vi "Get News.vi"(8 "error in":errorcluster, 11 "count":i32=10) -> (0 "error out":errorcluster, 3 "News":T1(array[cluster]))   [LabVIEW 2020, in "Full Featured MCP Server.lvlib"]
doc: "Returns the latest news of the market, newest first. News move prices: each item says what happened, which stocks it affects, the direction, and how far those stocks have moved since just before the news (affected: one entry per stock with its own move_since_percent), so you can judge whether it is already priced in. Part of an effect arrives at once, the rest builds up over the following minutes, and a first overreaction can partly reverse. Some items belong to a story that unfolds over minutes (a rumour, a launch date, an inquiry, a tender): the early items come before the big move, and how the story ends is uncertain."
uses:
  Full Featured MCP Server.lvlib
  Market/Market Mode.ctl
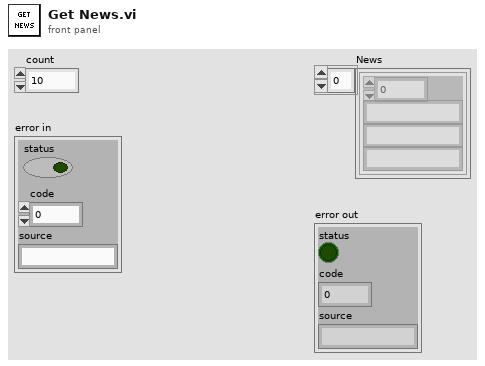
[diagram p1: front panel]
types:
  T1 = cluster{"age_seconds":i32, "headline":string, "direction":string, "affected":cluster{"name":string, "move_since_percent":dbl}[]}[]
  T2 = typedef "Full Featured MCP Server.lvlib/Market Mode.ctl" = enum16{"Get", "Init", "Advance", "Buy", "Sell"}
  T3 = typedef "Full Featured MCP Server.lvlib/Market State.ctl" = cluster{"tick":i32, "price history":dbl[][], "shock":dbl[], "momentum":dbl[], "nervousness":dbl[], "mood":dbl, "tension":dbl, "sector mood":dbl[], "news":T4[], "stories":cluster{"arc":i32, "step":i32, "due":i32, "stock":i32, "other":i32}[], "owned":i32[], "wallet":dbl}
  T4 = typedef "Full Featured MCP Server.lvlib/News Item.ctl" = cluster{"tick":i32, "headline":string, "stocks":i32[], "direction":string}
  T5 = cluster{"age_seconds":i32, "headline":string, "direction":string, "affected":cluster{"name":string, "move_since_percent":dbl}[]}
  T6 = cluster{"name":string, "move_since_percent":dbl}[]
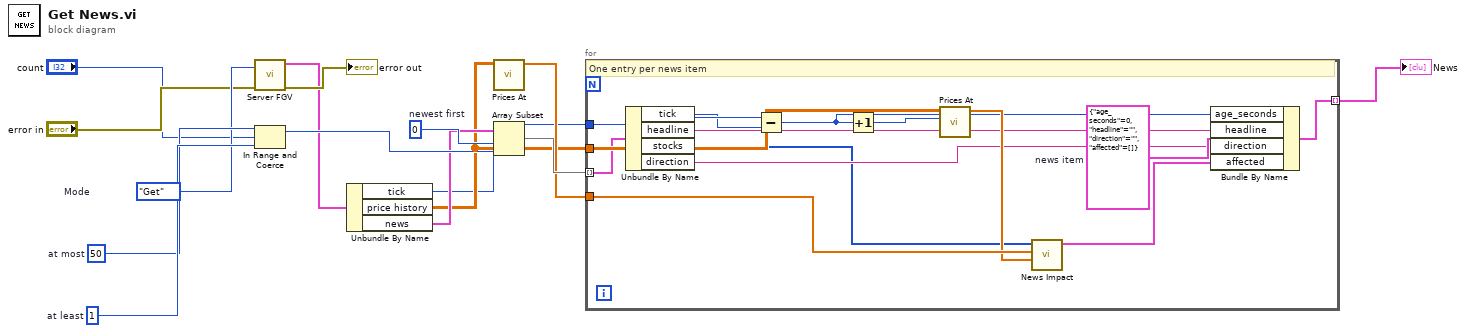
[diagram p0: block diagram]
diagram:
  w15 = 0  # newest first
  w10 = 1  # at least
  w9 = 50  # at most
  w3 = Market_Mode."Get"  # Mode
  n1 = call "Server FGV.vi"("Mode"=w3, "error in"="error in") -> ("error out"=→"error out":errorcluster, "market"=w4:T3)  [unwired: 7 in, 1 out]
  n2 = In Range and Coerce(upper limit=w9, x="count", lower limit=w10) -> (coerced(x)=w11:i32)  [unwired: 1 out]
  n3 = Unbundle By Name(w4) -> ("tick"=w6:i32, "price history"=w7:dbl[][], "news"=w8:T4[])
  n4 = call "Prices At.vi"("price history"=w7) -> ("prices"=w12:dbl[])  [unwired: 10 in]
  n5 = Array Subset(array=w8, index=w15, length=w11) -> (w13:T4[])
  n6 = for {
    tunnel: w6 -> [w21]
    tunnel: w7 -> [w24]
    tunnel: w13 -> [w16] mode=indexing
    tunnel: w12 -> [w26]
    tunnel: [w29] -> w14 mode=indexing
    w28 = T5 {"age_seconds"=0, "headline"="", "direction"="", "affected"=[]}  # news item
    # "One entry per news item"
    n7 = Unbundle By Name(w16) -> ("tick"=w17:i32, "headline"=w18:string, "stocks"=w19:i32[], "direction"=w20:string)
    n8 = Subtract(x=w21, y=w17) -> (x-y=w22:i32)
    n9 = Increment(x=w22) -> (x+1=w23:i32)
    n10 = call "Prices At.vi"("seconds ago"=w23, "price history"=w24) -> ("prices"=w25:dbl[])  [unwired: 9 in]
    n11 = call "News Impact.vi"("prices before"=w25, "prices now"=w26, "stocks"=w19) -> ("affected"=w27:T6)  [unwired: 8 in]
    n12 = Bundle By Name(cluster=w28, "age_seconds"=w22, "headline"=w18, "direction"=w20, "affected"=w27) -> (w29:T5)
  }
  "News" <- w14
